vi "Lab1_task2.vi"() -> ()   [LabVIEW 2022 SP3]
uses:
  <vilib>/Utility/file.llb/Read Delimited Spreadsheet (I64).vi
  <vilib>/Utility/file.llb/Write Delimited Spreadsheet (DBL).vi
panel:
  in  "file path (dialog if empty) 2":path
  out "all rows":i64[][](array[numeric])
  in  "file path (dialog if empty)":path
  out "Array":dbl[](array[numeric]) format="%.9g"
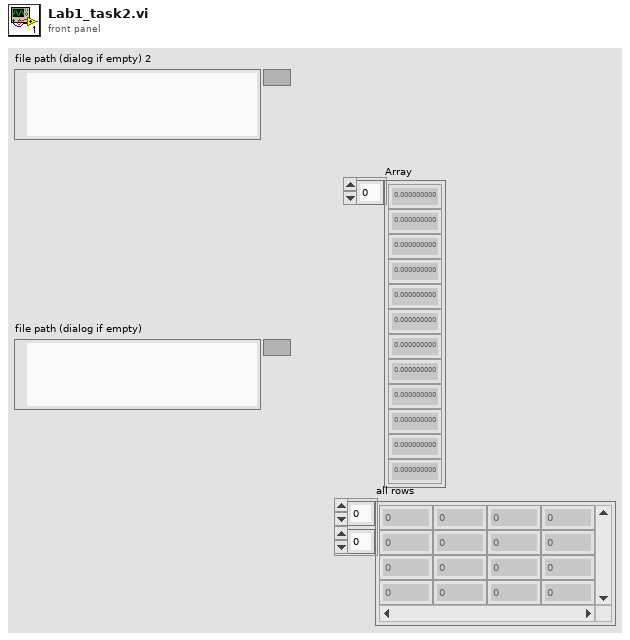
[diagram p1: front panel]
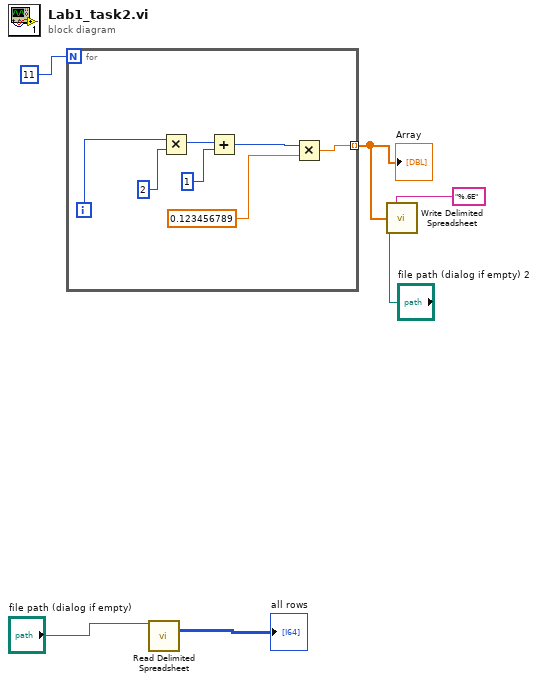
[diagram p0: block diagram]
diagram:
  n1 = for {
    N: 11 -> [_]
    tunnel: [w8] -> w3 mode=indexing
    i -> [w13]
    n2 = Multiply(x=w13, y=2) -> (x*y=w11:i32)
    n3 = Add(x=w11, y=1) -> (x+y=w7:i32)
    n4 = Multiply(x=w7, y=0.123456789) -> (x*y=w8:dbl)
  }
  "Array" <- w3
  n5 = call-poly <vilib>:"Read Delimited Spreadsheet.vi"("file path (dialog if empty)"="file path (dialog if empty)") -> ("all rows"=→"all rows":i64[][])  [unwired: 9 in, 5 out]
  n6 = call-poly <vilib>:"Write Delimited Spreadsheet.vi"("file path (dialog if empty)"="file path (dialog if empty) 2", "format (%.3f)"="%.6E", "1D data"=w3) -> ()  [unwired: 11 in, 2 out]
